vi "user32 GetAncestor.vi"(0 "hwnd":u64, 5 "gaFlags":u32=2, 11 "error in":errorcluster) -> (4 "ancestor":u64, 15 "error out":errorcluster)   [LabVIEW 2020, in "RemoteVI.lvlib"]
doc: "Returns an ancestor of the window hwnd through user32.dll GetAncestor (stdcall, called in any thread). gaFlags 2 GA_ROOT (default) gives the top-level window hwnd is part of, e.g. the dialog a focused edit control belongs to; 1 GA_PARENT the parent, 3 GA_ROOTOWNER the root window of the owner chain. ancestor is 0 when hwnd is not a window. When error in carries an error the DLL is not called. Generated by scripts\\Build Win32 Wrappers.vi - do not edit by hand, rebuild it."
uses:
  RemoteVI.lvlib
  user32.dll
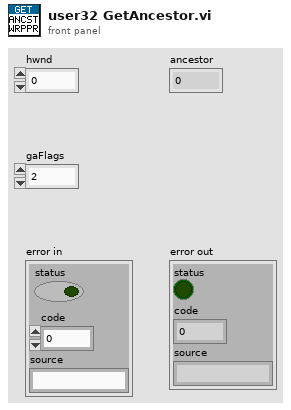
[diagram p1: front panel]
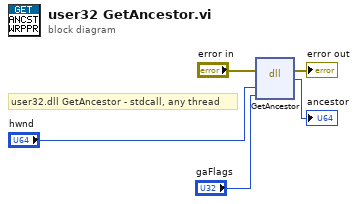
[diagram p0: block diagram]
diagram:
  # "user32.dll GetAncestor - stdcall, any thread"
  n1 = dll-call lib="user32.dll" fn="GetAncestor"(error in="error in", "hwnd"="hwnd", "gaFlags"="gaFlags") -> (error out=→"error out":errorcluster, →"ancestor":u64)  [unwired: 4 in, 1 out]
